vi "GetCachedFeed.vi"(8 "error in (no error)":errorcluster, 9 "default URL":string, 10 "feed GUID":string) -> (0 "error out":errorcluster, 2 "cache found":bool, 3 "Feed":refnum<class "Feed.lvclass">)   [LabVIEW 2023, in "GettingStartedWindow.lvlib" / "Feed_link.lvclass"]
uses:
  <resource>/modes/FRC/GSW/Classes/Feed_link/Feed_link.lvclass
  <vilib>/NI_RSS/Feed/Feed.lvclass
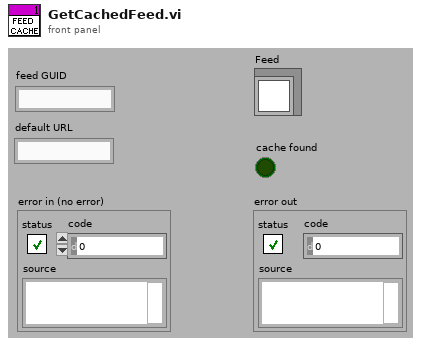
[diagram p1: front panel]
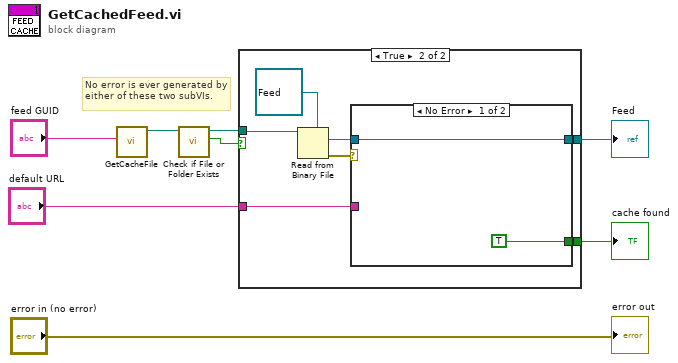
[diagram p0: block diagram]
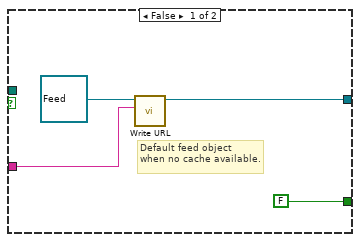
[diagram p2: hidden frame]
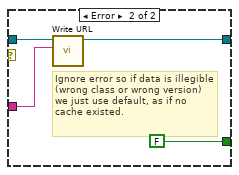
[diagram p3: hidden frame]
diagram:
  # "No error is ever generated by\neither of these two subVIs."
  n1 = call <resource>:"GetCacheFile.vi"("feed GUID"="feed GUID") -> ("cache file"=w7:path)  [unwired: 1 in, 9 out]
  n2 = call <vilib>:"Check if File or Folder Exists.vi"("path"=w7) -> ("file or folder exists?"=w6:bool, "dup path"=w5:path)  [unwired: 1 in, 8 out]
  n3 = case shown="True" w6 {
    tunnel: w5 -> [_ w19]
    tunnel: [w11 w15] -> w4
    tunnel: "default URL" -> [w10 w13]
    tunnel: [FALSE w16] -> w1
    frame False {
      # "Default feed object\nwhen no cache available."
      n4 = call <vilib>:"Write URL.vi"("URL"=w10, "Feed.lvclass in"=refnum<class "Feed.lvclass"> refnum ("Feed")) -> ("Feed.lvclass out"=w11:refnum<class "Feed.lvclass">)  [unwired: 1 in, 8 out]
    }
    frame True {
      n5 = Read from Binary File(5:refnum<class "Feed.lvclass"> refnum ("Feed"), 11:w19) -> (0:w17:errorcluster, 2:w14:refnum<class "Feed.lvclass">)  [unwired: 1 in, 5 out]
      n6 = case shown="No Error" w17 {
        tunnel: [TRUE FALSE] -> w16
        tunnel: [w20 w24] -> w15
        tunnel: w14 -> [w20 w22]
        tunnel: w13 -> [_ w23]
        frame No Error {
        }
        frame Error {
          # "Ignore error so if data is illegible\n(wrong class or wrong version)\nwe just use default, as if no\ncache existed."
          n7 = call <vilib>:"Write URL.vi"("URL"=w23, "Feed.lvclass in"=w22) -> ("Feed.lvclass out"=w24:refnum<class "Feed.lvclass">)  [unwired: 1 in, 8 out]
        }
      }
    }
  }
  "Feed" <- w4
  "cache found" <- w1
  "error out" <- "error in (no error)"
